vi "Convert Replace Column to Options.vi"(11 "Replace Column":T1) -> (1 "Visible?":bool, 3 "Replace Options":string[](array[string]))   [LabVIEW 2020, in "VI Properties Editor.lvlib"]
doc: "Converts <B>Replace Column</B> to a list of <B>Replace Options</B>."
uses:
  VI Properties Editor.lvlib
  CTLs/Replace Column.ctl
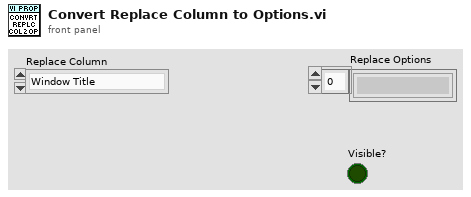
[diagram p1: front panel]
types:
  T1 = typedef "VI Properties Editor.lvlib/Replace Column.ctl" = enum16{"Window Title", "Description", "Help Path", "Help Tag", "Custom Title?", "Help URL", "Help Type", "Inlined?", "Allow debugging?", "Auto error handling?", "Run when opened?", "Suspend when called?", "Reentrancy", "Priority", "Preferred Exec System", "Control Label", "Control Caption", "Control Description", "Control Tip Strip"}
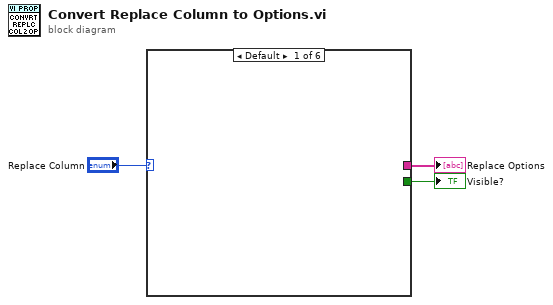
[diagram p0: block diagram]
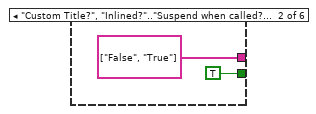
[diagram p2: hidden frame]
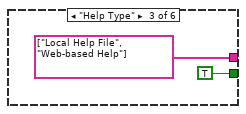
[diagram p3: hidden frame]
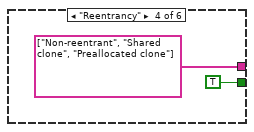
[diagram p4: hidden frame]
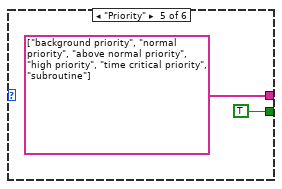
[diagram p5: hidden frame]
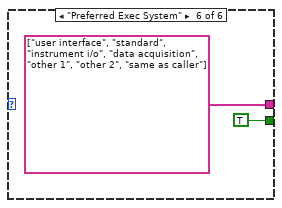
[diagram p6: hidden frame]
diagram:
  n1 = case shown="Default" "Replace Column" {
    tunnel: [_ string[] ["False", "True"] string[] ["Local Help File", "Web-based Help"] string[] ["Non-reentrant", "Shared clone", "Preallocated clone"] string[] ["background priority", "normal priority", "above normal priority", "high priority", "time critical priority", "subroutine"] string[] ["user interface", "standard", "instrument i/o", "data acquisition", "other 1", "other 2", "same as caller"]] -> w2
    tunnel: [_ TRUE ("Visible") TRUE ("Visible") TRUE ("Visible") TRUE ("Visible") TRUE ("Visible")] -> w1
    frame Default {
    }
    frame "Custom Title?", "Inlined?".."Suspend when called?" {
    }
    frame "Help Type" {
    }
    frame "Reentrancy" {
    }
    frame "Priority" {
    }
    frame "Preferred Exec System" {
    }
  }
  "Replace Options" <- w2
  "Visible?" <- w1
